vi "New RegReadExtLong Command.vi"(0 "RFFE RegReadExtLong Command in":refnum<class "RFFE RegReadExtLong Command.lvclass">, 1 "Alias":string, 5 "Slave Address":T2=12 format="%02x", 7 "Register Address":T1 format="%02x", 9 "Byte Count":i32=1, 11 "error in (no error)":errorcluster) -> (4 "RFFE RegReadExtLong Command out":refnum<class "RFFE RegReadExtLong Command.lvclass">, 15 "error out":errorcluster)   [LabVIEW 2018, in "MIPI RFFE API.lvlib" / "RFFE RegReadExtLong Command.lvclass"]
uses:
  RFFE RegReadExtLong Command.lvclass
  C:/Users/semoore/Projects/mipi-rffe-labview-oop/RegReadExt/RFFE RegReadExt Command.lvclass
  Slave Address.ctl
  Register Address.ctl
  RegReadExt/RFFE RegReadExt Command.lvclass
  MIPI RFFE API.lvlib
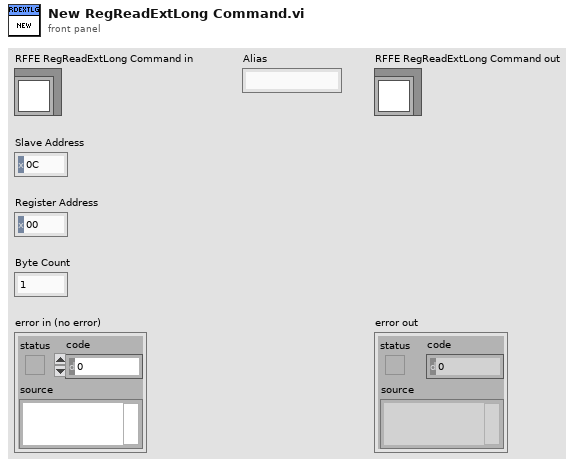
[diagram p1: front panel]
types:
  T1 = typedef "MIPI RFFE API.lvlib/Register Address.ctl" = u16
  T2 = typedef "MIPI RFFE API.lvlib/Slave Address.ctl" = u8
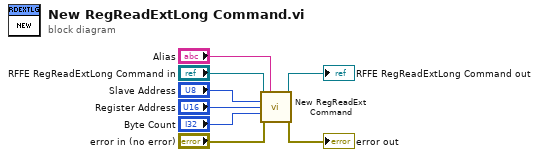
[diagram p0: block diagram]
diagram:
  n1 = call "New RegReadExt Command.vi"("RFFE RegReadExt Command in"="RFFE RegReadExtLong Command in", "Alias"="Alias", "Slave Address"="Slave Address", "Register Address"="Register Address", "Byte Count"="Byte Count", "error in (no error)"="error in (no error)") -> ("RFFE RegReadExt Command out"=→"RFFE RegReadExtLong Command out":refnum<class "RFFE RegReadExtLong Command.lvclass">, "error out"=→"error out":errorcluster)  [unwired: 8 in]
